vi "Material Theme Editor.vi"() -> ()   [LabVIEW 2021]
doc: "Import Material m3 JSON files to see the color scheme in LabVIEW.\n\nActions: +\n- Color Scheme: view and change colors for the theme mode +\n- Palette: see the palette color scales +\n- Text: see the text from the JSON file +\n- Buttons: see examples of the application to material button components - they can also be right clicked and copied so they can be directly pasted on an open front panel +\n\nOther options: +\n- Save the changes made in the editor (or save to a new file) +\n- Preview the theme on a lot of different front panel UI components +\n- See the overall colors of the palette and give ability to import into <i>User Colors</i>\n\n<b>Note:</b> if using the legacy XML files from earlier versions of the tool, they can be converted to the json format directly (assuming the original source doesn't exist still)\n\n<b>Code Developed By:</b> +\nDaniel Coons +\nTechnology Service Corporation +\nwww.tsc.com/atcs"
uses:
  Material Theme/Material Theme.lvclass
  _theme-editor/Theme Config/Theme Config.lvclass/Theme Config.ctl
  Material-Scheme/Material-Scheme.lvclass/Material-Scheme.ctl
  Material-Scheme/View-User Colors.vi
  Material-Scheme/Material-Scheme.lvclass
  Material-Palette/Material-Palette.lvclass
  user32.dll
  <vilib>/Utility/traverseref.llb/VI Scripting - Traverse.lvlib
  <vilib>/Utility/traverseref.llb/TRef TravTarget.ctl
  _theme-editor/Theme Config/Theme Config.lvclass
panel:
  in  "palette":bool
  in  "File Interaction":enum32{"load--buton", "convert--buton"}(radio)
  in  "tabs":enum32{"color", "palette", "json", "buttons"}(radio)
  in  "preview":bool
  in  "close":bool
  out "header":bool
  in  "save":bool
  in  "Theme Mode":u16(ring) items=["Light Theme", "Light Medium Contrast", "Light High Contrast", "Dark Theme", "Dark Medium Contrast", "Dark High Constrast"]
  in  "Tab Control":T1(tab)
  out "material JSON output":string
  in  "Color Level":u16(ring) items=["Primary", "Secondary", "Tertiary", "Error", "Primary Fixed", "Secondary Fixed", "Tertiary Fixed"]
  in  "Tab Control file":enum32{"load", "convert"}(tab)
  in  "json file path":path caption="Material Theme JSON File"
  in  "LabVIEW material theme":path
  # "Load a JSON M3 theme file from Google to \nview and edit the scheme."
  # "Can be generated through Figma or at:   https://material-foundation.github.io/material-theme-builder/<Material Website>"
  # "Load a TSC Material Theme legacy XML file to see modes\nand palette colors and convert to JSON format for long-term\nsupport."
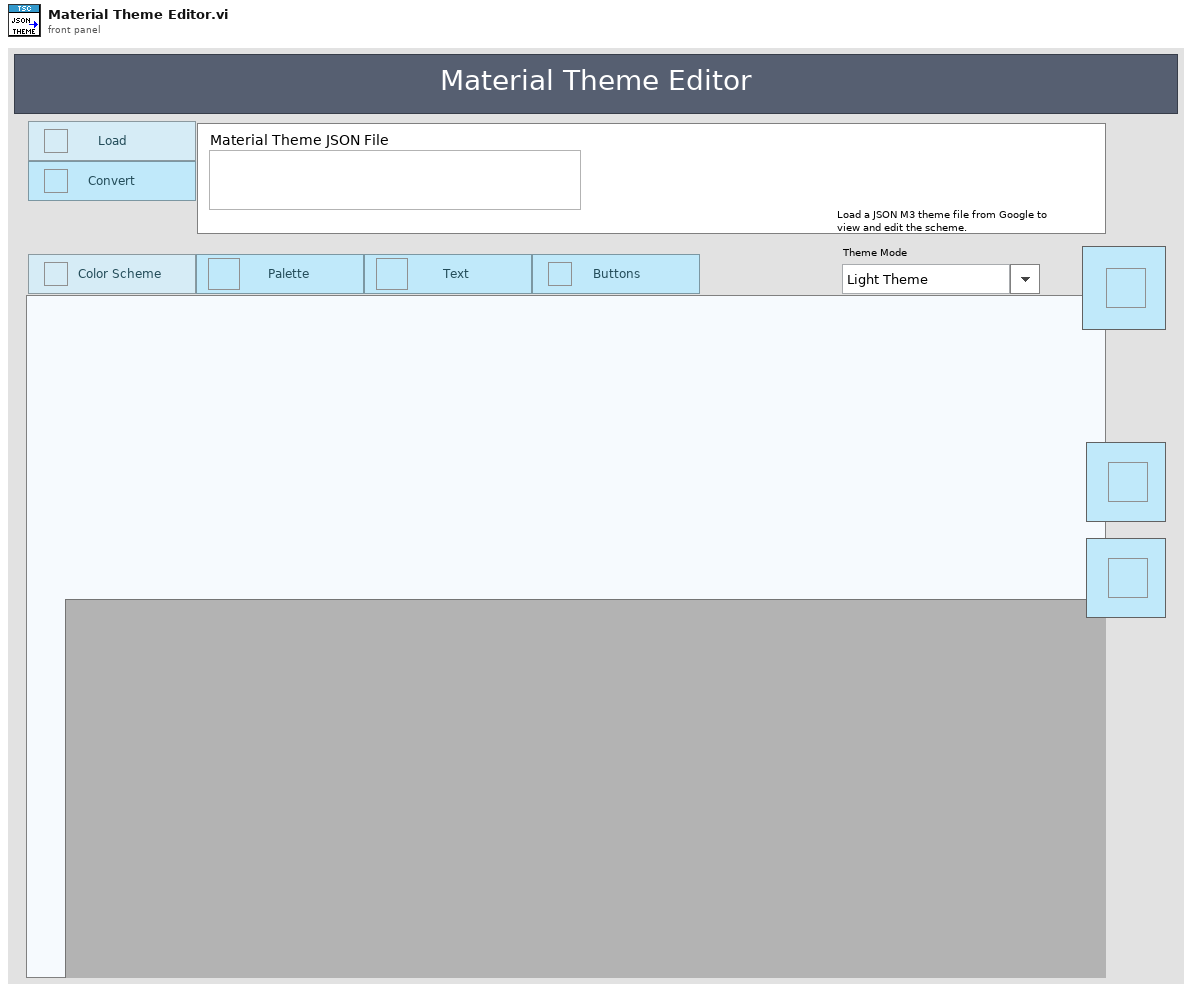
[diagram p1: front panel]
types:
  T1 = enum32{"Color Scheme", "Palette Variations", "JSON String", "buttons"}
  T2 = typedef "TRef TravTarget.ctl" = enum16{"FP", "BD", "Other"}
  T3 = enum16{"open", "replace", "create", "open or create", "replace or create", "replace or create with confirmation"}
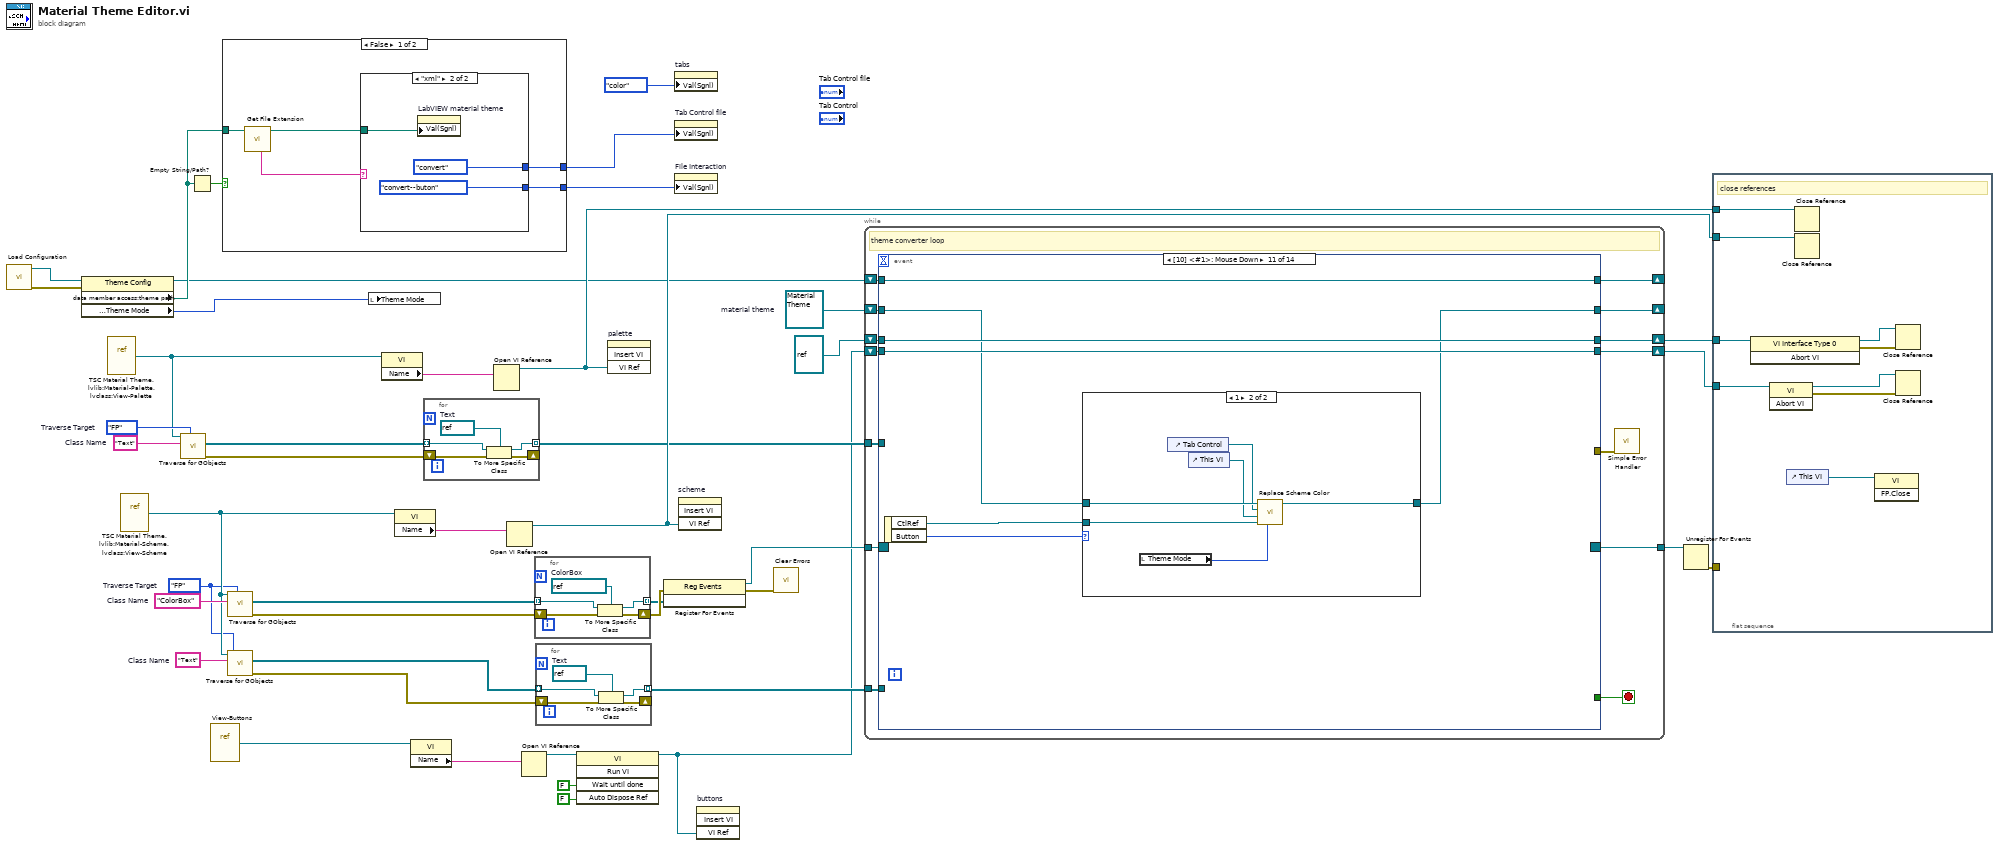
[diagram p0: block diagram]
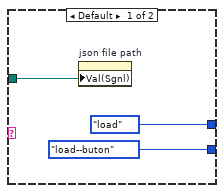
[diagram p2: hidden frame]
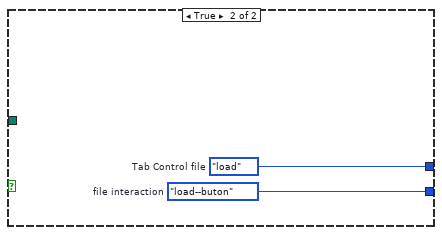
[diagram p3: hidden frame]
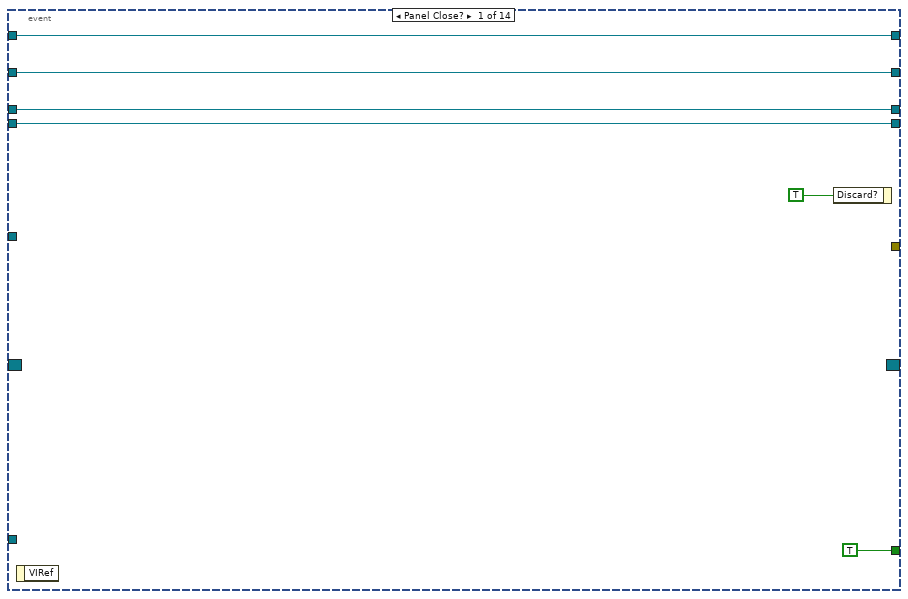
[diagram p4: hidden frame]
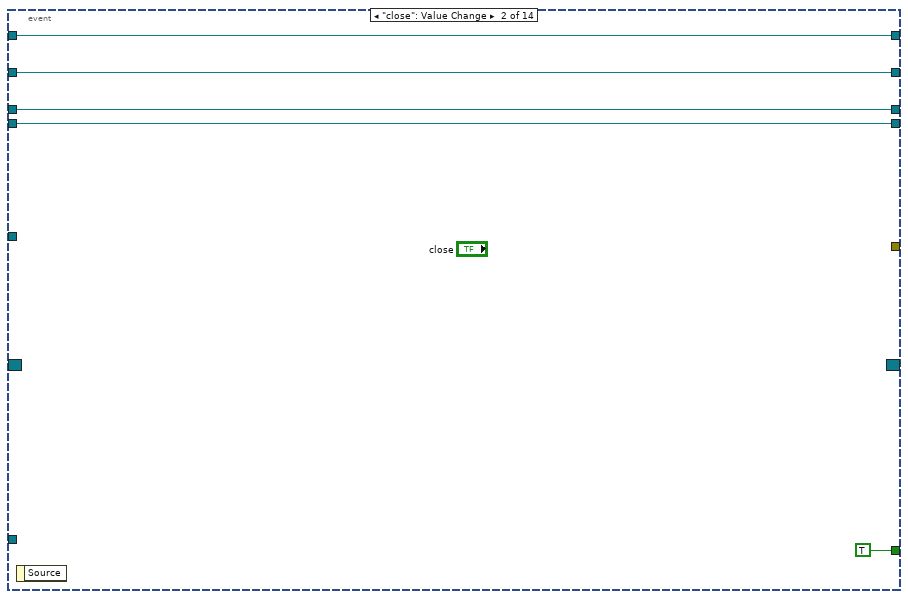
[diagram p5: hidden frame]
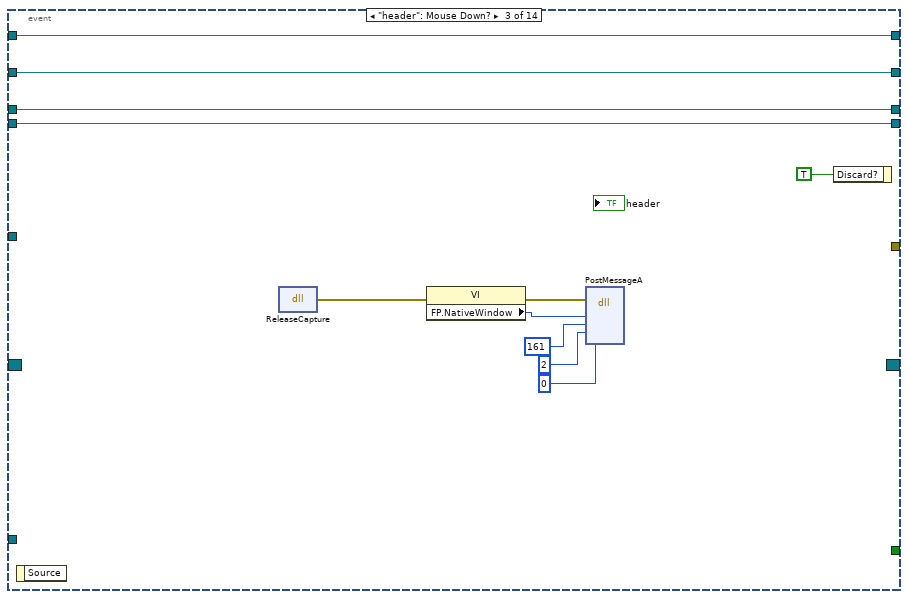
[diagram p6: hidden frame]
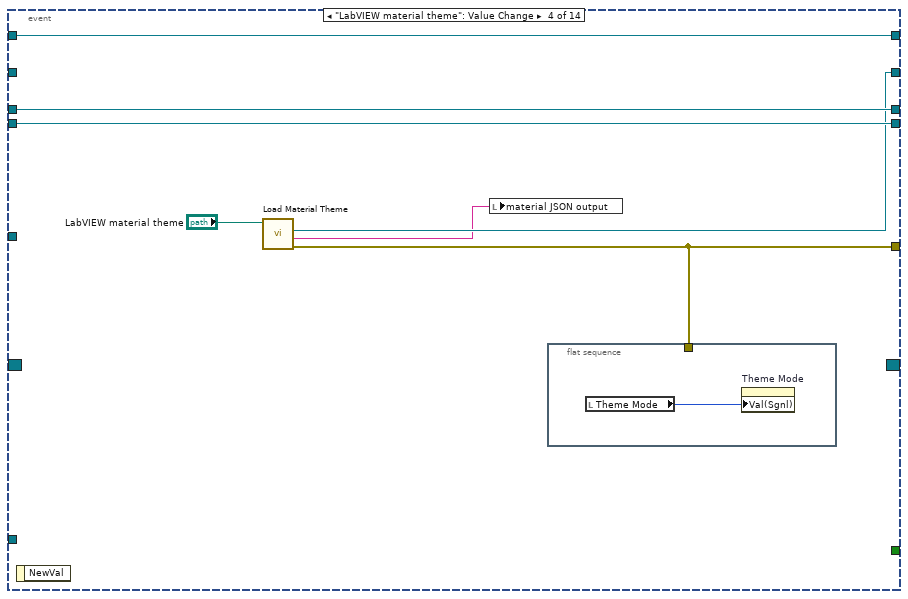
[diagram p7: hidden frame]
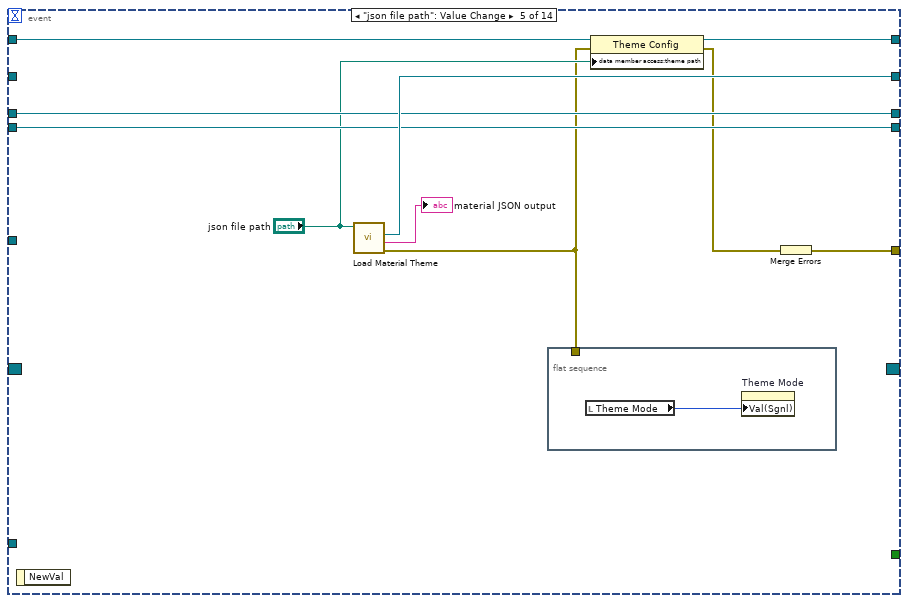
[diagram p8: hidden frame]
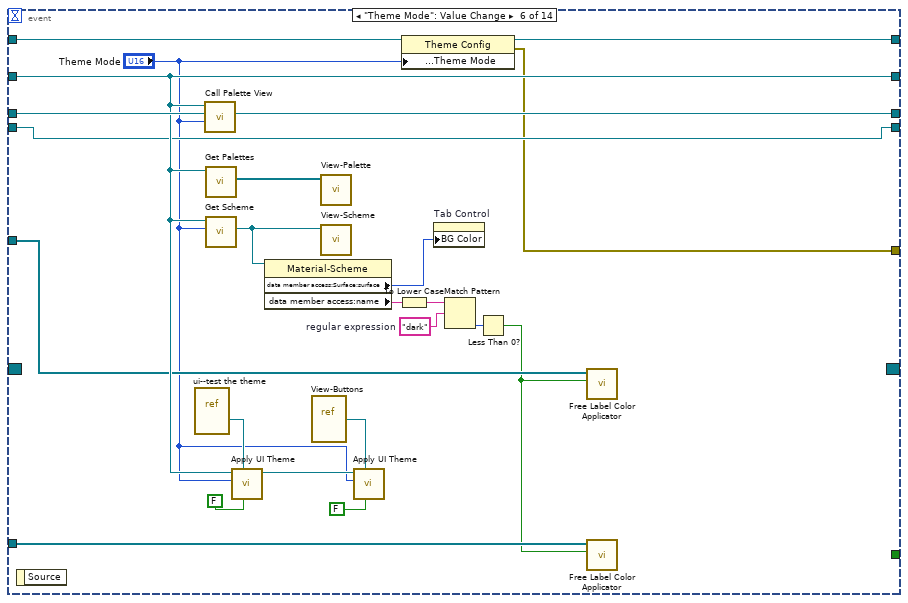
[diagram p9: hidden frame]
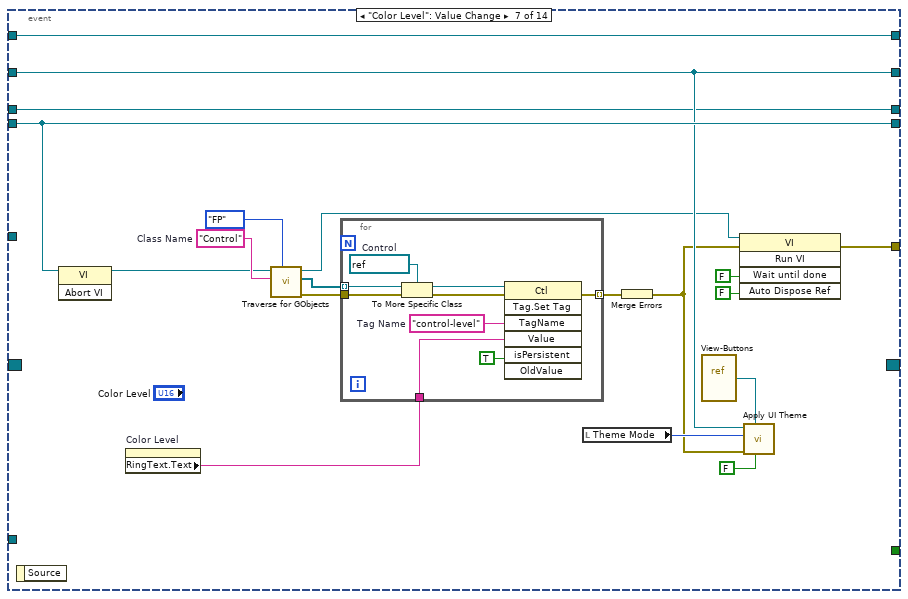
[diagram p10: hidden frame]
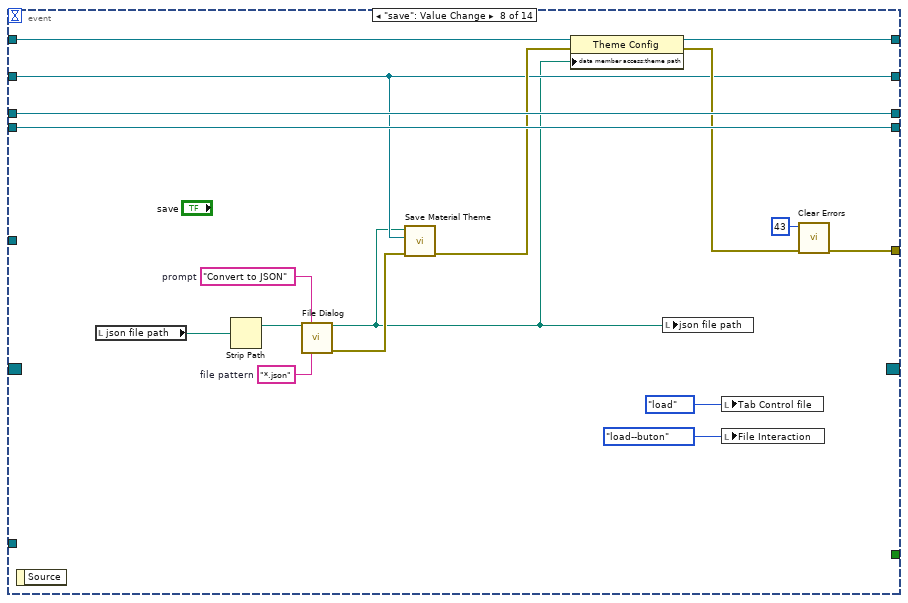
[diagram p11: hidden frame]
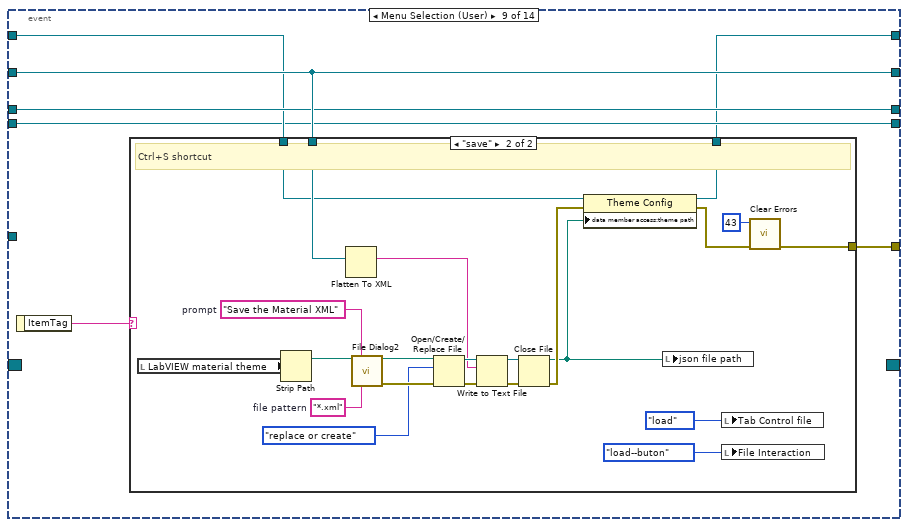
[diagram p12: hidden frame]
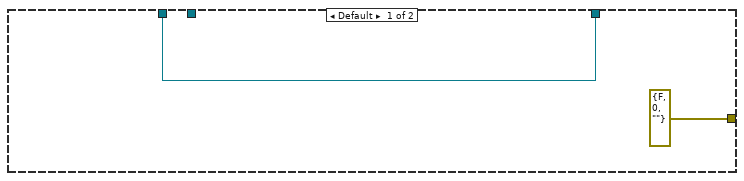
[diagram p13: hidden frame]
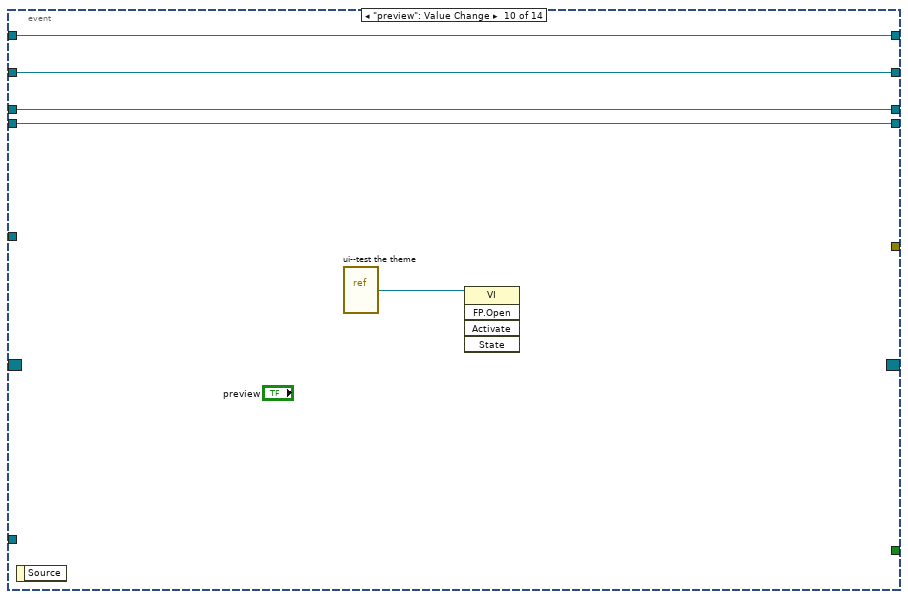
[diagram p14: hidden frame]
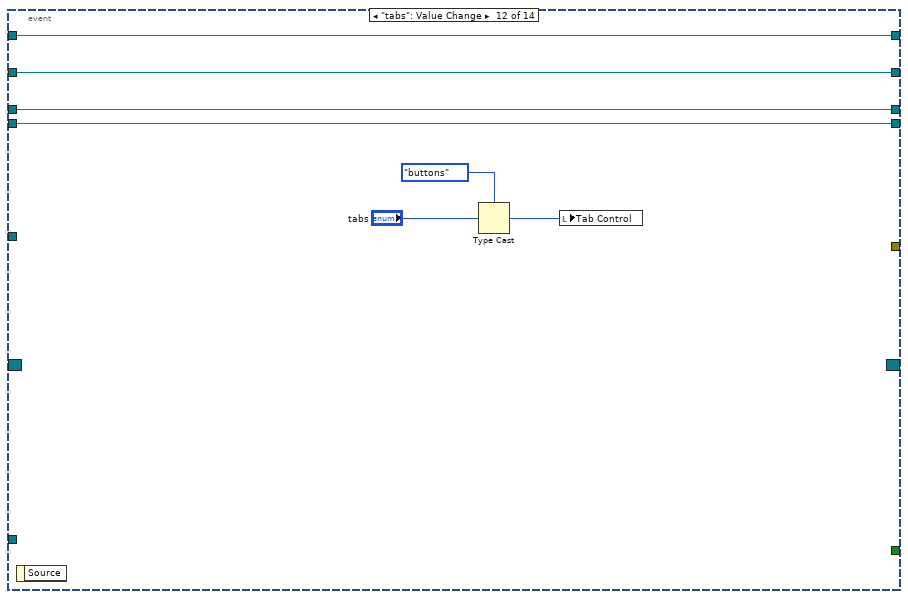
[diagram p16: hidden frame]
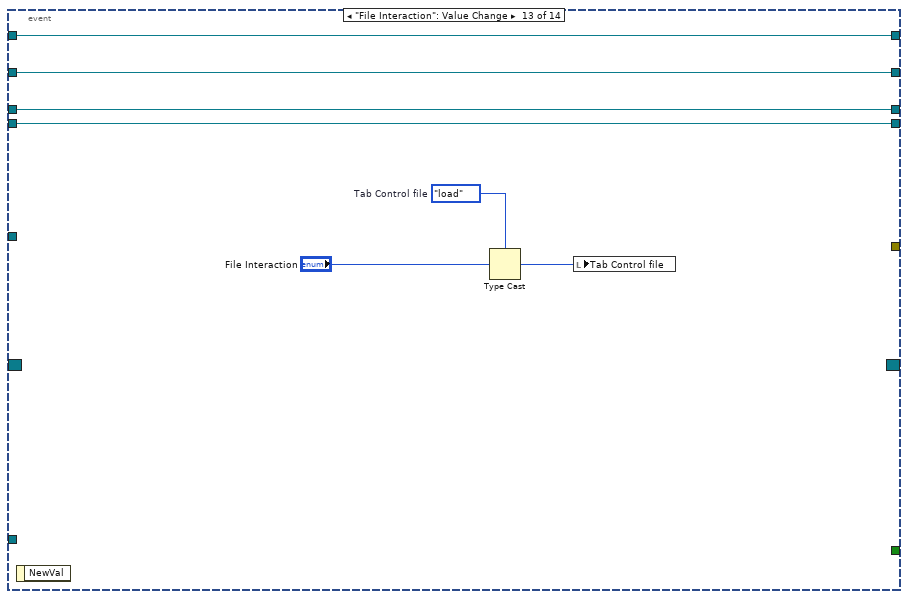
[diagram p17: hidden frame]
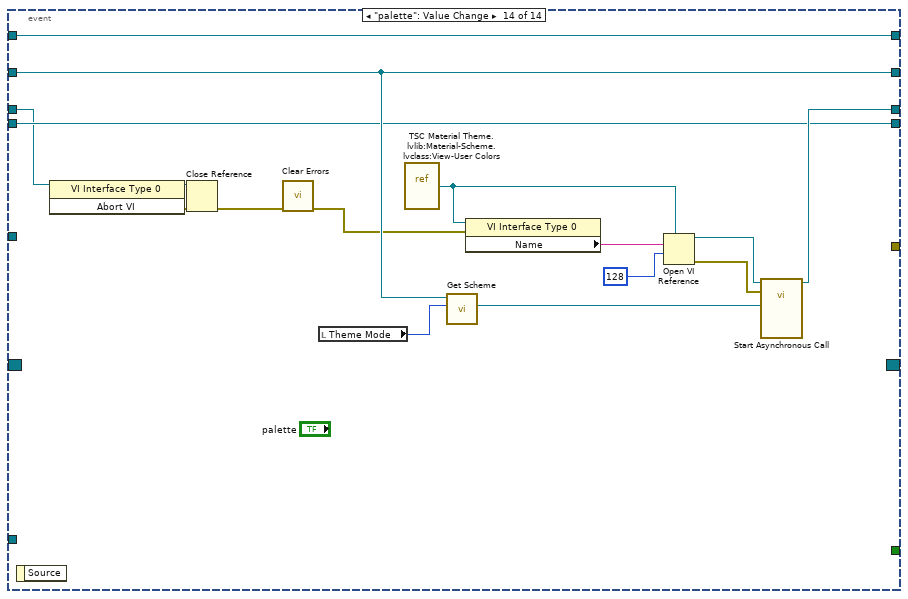
[diagram p18: hidden frame]
diagram:
  w24 = "Text"  # Class Name
  w27 = "Text"  # Class Name
  w28 = TRef_TravTarget."FP"  # Traverse Target
  w30 = refnum<class "Material Theme.lvclass"> refnum  # material theme
  w36 = "ColorBox"  # Class Name
  w22 = TRef_TravTarget."FP"  # Traverse Target
  n1 = call "Load Configuration.vi"() -> ("error out"=w10:errorcluster, "Theme Config out"=w9:refnum<class "Theme Config.lvclass">)  [unwired: 10 in]
  n2 = property class="Theme Config"(reference=w9, error in=w10) -> (reference out=w6:refnum<class "Theme Config.lvclass">, "data member access:theme path"=w8:path, "data member access:Theme Mode"=w3:u16)  [unwired: 1 out]
  n3 = vi-ref "TSC Material Theme.lvlib:Material-Palette.lvclass:View-Palette.vi"() -> (w7:refnum<vi>)
  n4 = vi-ref "TSC Material Theme.lvlib:Material-Scheme.lvclass:View-Scheme.vi"() -> (w23:refnum<vi>)
  n5 = call <vilib>:"Traverse for GObjects.vi"("Traverse Target"=w28, "Class Name"=w27, "VI Refnum"=w7) -> ("error out"=w41:errorcluster, "References"=w26:refnum<vi>[])  [unwired: 5 in, 2 out]
  n6 = Empty String/Path?(string/path=w8) -> (empty?=w29:bool)
  n7 = vi-ref "View-Buttons.vi"() -> (w17:refnum<vi>)
  n8 = case shown="False" w29 {
    tunnel: w8 -> [w49 _]
    tunnel: [w48 w56] -> w2
    tunnel: [w47 w57] -> w1
    frame False {
      n9 = call <vilib>:"Get File Extension.vi"("file"=w49) -> ("dup file"=w46:path, "unmodified file extension"=w45:string)  [unwired: 6 in, 3 out]
      n10 = case shown="\"xml\"" w45 {
        tunnel: w46 -> [w52 w55]
        tunnel: [enum32{"load--buton", "convert--buton"}."load--buton" ("Value (Signaling)") enum32{"load--buton", "convert--buton"}."convert--buton" ("Value (Signaling)")] -> w48
        tunnel: [enum32{"load", "convert"}."load" ("Tab Control file") enum32{"load", "convert"}."convert" ("Tab Control file")] -> w47
        frame Default {
          n11 = property on="json file path" class="Path"("Val(Sgnl)"=w52) -> ()  [unwired: 2 in, 2 out]
        }
        frame "xml" {
          n12 = property on="LabVIEW material theme" class="Path"("Val(Sgnl)"=w55) -> ()  [unwired: 2 in, 2 out]
        }
      }
    }
    frame True {
      w56 = enum32{"load--buton", "convert--buton"}."load--buton"  # file interaction
      w57 = enum32{"load", "convert"}."load"  # Tab Control file
    }
  }
  n13 = call <vilib>:"Traverse for GObjects.vi"("Traverse Target"=w22, "Class Name"=w36, "VI Refnum"=w23) -> ("error out"=w44:errorcluster, "References"=w34:refnum<vi>[])  [unwired: 5 in, 2 out]
  n14 = call <vilib>:"Traverse for GObjects.vi"("Traverse Target"=w22, "Class Name"=w24, "VI Refnum"=w23) -> ("error out"=w40:errorcluster, "References"=w21:refnum<vi>[])  [unwired: 5 in, 2 out]
  n15 = local write "Theme Mode"(w3) -> ()
  n16 = property class="VI"(reference=w7) -> ("Name"=w39:string)  [unwired: 1 in, 2 out]
  n17 = property class="VI"(reference=w23) -> ("Name"=w38:string)  [unwired: 1 in, 2 out]
  n18 = property class="VI"(reference=w17) -> ("Name"=w16:string)  [unwired: 1 in, 2 out]
  n19 = for {
    tunnel: w26 -> [w59] mode=indexing
    shift-right: [w61] -> _
    shift-left: w41 -> [w62]
    tunnel: [w58] -> w25 mode=indexing
    w60 = refnum<vi> refnum  # Text
    n20 = To More Specific Class(target class=w60, reference=w59, error in=w62) -> (specific class reference=w58:refnum<vi>, error out=w61:errorcluster)
  }
  n21 = Open VI Reference(vi path=w39) -> (vi reference=w37:refnum<vi>)  [unwired: 5 in, 1 out]
  n22 = Open VI Reference(vi path=w38) -> (vi reference=w33:refnum<vi>)  [unwired: 5 in, 1 out]
  n23 = Open VI Reference(vi path=w16) -> (vi reference=w18:refnum<vi>)  [unwired: 5 in, 1 out]
  n24 = for {
    tunnel: w34 -> [w64] mode=indexing
    shift-right: [w66] -> w43
    shift-left: w44 -> [w67]
    tunnel: [w63] -> w32 mode=indexing
    w65 = refnum<vi> refnum  # ColorBox
    n25 = To More Specific Class(target class=w65, reference=w64, error in=w67) -> (specific class reference=w63:refnum<vi>, error out=w66:errorcluster)
  }
  n26 = for {
    tunnel: w21 -> [w69] mode=indexing
    shift-right: [w71] -> _
    shift-left: w40 -> [w72]
    tunnel: [w68] -> w20 mode=indexing
    w70 = refnum<vi> refnum  # Text
    n27 = To More Specific Class(target class=w70, reference=w69, error in=w72) -> (specific class reference=w68:refnum<vi>, error out=w71:errorcluster)
  }
  n28 = invoke class="VI" method="Run VI"(reference=w18, "Wait until done"=FALSE ("Wait Until Done"), "Auto Dispose Ref"=FALSE ("Auto Dispose Reference")) -> (reference out=w13:refnum<vi>)  [unwired: 2 in, 4 out]
  n29 = invoke on="palette" class="SubPnl" method="Insert VI"("VI Ref"=w37) -> ()  [unwired: 3 in, 4 out]
  n30 = register-events(error in=w43, w32) -> (reference out=w35:refnum<event-registration>, error out=w42:errorcluster)  [unwired: 1 in]
  n31 = property on="tabs" class="RadioBtnsControl (strict)"("Val(Sgnl)"=enum32{"color", "palette", "json", "buttons"}."color" ("Value (Signaling)")) -> ()  [unwired: 2 in, 2 out]
  n32 = property on="Tab Control file" class="TabCtl (strict)"("Val(Sgnl)"=w1) -> ()  [unwired: 2 in, 2 out]
  n33 = property on="File Interaction" class="RadioBtnsControl (strict)"("Val(Sgnl)"=w2) -> ()  [unwired: 2 in, 2 out]
  n34 = invoke on="scheme" class="SubPnl" method="Insert VI"("VI Ref"=w33) -> ()  [unwired: 3 in, 4 out]
  n35 = invoke on="buttons" class="SubPnl" method="Insert VI"("VI Ref"=w13) -> ()  [unwired: 3 in, 4 out]
  n36 = call <vilib>:"Clear Errors.vi"("error in (no error)"=w42) -> ()  [unwired: 5 in, 2 out]
  n37 = while {
    shift-right: [w84] -> _
    shift-left: w30 -> [w83]
    tunnel: w35 -> [w82]
    tunnel: [w81] -> w31
    tunnel: w25 -> [w80]
    tunnel: w20 -> [w79]
    shift-right: [w77] -> w12
    shift-left: refnum<vi> refnum -> [w76]
    shift-right: [w74] -> _
    shift-left: w6 -> [w75]
    shift-right: [w73] -> w4
    shift-left: w13 -> [w78]
    stop <- w85 stop-if-true
    # "theme converter loop"
    n38 = event shown="[10] <#1>: Mouse Down" {
      selector: w82 -> [_ _ _ _ _ _ _ _ _ _ _ _ _ _]
      dyn-events: [_ _ _ _ _ _ _ _ _ _ _ _ _ _] -> w81
      timeout: _ -> [_ _ _ _ _ _ _ _ _ _ _ _ _ _]
      tunnel: [TRUE TRUE _ _ _ _ _ _ _ _ _ _ _ _] -> w85
      tunnel: [w90 w97 w101 w110 w125 w137 w156 w182 w201 w231 w232 w252 w258 w275] -> w84
      tunnel: w83 -> [w90 w97 w101 _ _ w137 w156 w182 w201 w231 w233 w252 w258 w275]
      tunnel: [_ _ _ w111 w126 w128 w162 w185 w202 _ _ _ _ _] -> w86
      tunnel: w80 -> [_ _ _ _ _ w132 _ _ _ _ _ _ _ _]
      tunnel: w79 -> [_ _ _ _ _ w141 _ _ _ _ _ _ _ _]
      tunnel: w78 -> [w87 w93 w98 w113 w122 w133 w167 w187 w197 w227 w235 w246 w255 w265]
      tunnel: [w89 w95 w100 w115 w124 w136 w152 w190 w199 w229 w237 w248 w257 w267] -> w77
      tunnel: w76 -> [w89 w95 w100 w115 w124 w138 w152 w190 w199 w229 w237 w248 w257 w262]
      tunnel: w75 -> [w88 w94 w99 w114 w123 w134 w151 w189 w198 w228 w236 w247 w256 w266]
      tunnel: [w88 w94 w99 w114 w121 w130 w151 w188 w196 w228 w236 w247 w256 w266] -> w74
      tunnel: [w87 w93 w98 w113 w122 w133 w167 w187 w197 w227 w235 w246 w255 w265] -> w73
      event Panel Close? {
        n39 = event-data() -> ()  [unwired: 1 in, 1 out]
        n40 = event-data("Discard?"=TRUE) -> ()  [unwired: 1 in, 1 out]
      }
      event "close": Value Change {
        n41 = event-data() -> ()  [unwired: 1 in, 1 out]
      }
      event "header": Mouse Down? {
        n42 = event-data() -> ()  [unwired: 1 in, 1 out]
        n43 = dll-call lib="user32.dll" fn="ReleaseCapture"() -> (error out=w108:errorcluster)  [unwired: 4 in, 1 out]
        n44 = property class="VI"(error in=w108) -> (error out=w107:errorcluster, "FP.NativeWindow"=w102:u64)  [unwired: 1 in, 1 out]
        n45 = dll-call lib="user32.dll" fn="PostMessageA"(error in=w107, "hWnd"=w102, "Msg"=161, "wParam"=2, "lParam"=0) -> ()  [unwired: 7 in, 2 out]
        n46 = event-data("Discard?"=TRUE) -> ()  [unwired: 1 in, 1 out]
      }
      event "LabVIEW material theme": Value Change {
        n47 = event-data() -> ()  [unwired: 1 in, 1 out]
        n48 = call "Load Material Theme.vi"("file path"="LabVIEW material theme") -> ("error out"=w111:errorcluster, "text"=w109:string, "Theme"=w110:refnum<class "Material Theme.lvclass">)  [unwired: 8 in]
        n49 = local write "material JSON output"(w109) -> ()
        n50 = flat-sequence {
          tunnel: w111 -> [_]
          frame #0 {
            n51 = local read "Theme Mode"() -> (w116:u16)
            n52 = property on="Theme Mode" class="Ring (strict)"("Val(Sgnl)"=w116) -> ()  [unwired: 2 in, 2 out]
          }
        }
      }
      event "json file path": Value Change {
        n53 = event-data() -> ()  [unwired: 1 in, 1 out]
        n54 = call "Load Material Theme.vi"("file path"="json file path") -> ("error out"=w119:errorcluster, "text"=→"material JSON output":string, "Theme"=w125:refnum<class "Material Theme.lvclass">)  [unwired: 8 in]
        n55 = flat-sequence {
          tunnel: w119 -> [_]
          frame #0 {
            n56 = local read "Theme Mode"() -> (w127:u16)
            n57 = property on="Theme Mode" class="Ring (strict)"("Val(Sgnl)"=w127) -> ()  [unwired: 2 in, 2 out]
          }
        }
        n58 = property class="Theme Config"(reference=w123, error in=w119, "data member access:theme path"="json file path") -> (reference out=w121:refnum<class "Theme Config.lvclass">, error out=w118:errorcluster)
        n59 = Merge Errors(w118) -> (w126:errorcluster)
      }
      event "Theme Mode": Value Change {
        w144 = "dark"  # regular expression
        n60 = event-data() -> ()  [unwired: 1 in, 1 out]
        n61 = vi-ref "ui--test the theme.vi"() -> (w149:refnum<vi>)
        n62 = call "Call Palette View.vi"("Theme Mode"="Theme Mode", "VI ref in"=w138, "Material Theme"=w137) -> ("VI ref"=w136:refnum<vi>)  [unwired: 7 in, 1 out]
        n63 = call "Get Palettes.vi"("Material Theme in"=w137) -> ("Material-Palettes"=w150:refnum<class "Material-Palette.lvclass">[])  [unwired: 8 in, 2 out]
        n64 = call "Get Scheme.vi"("Theme"="Theme Mode", "Material Theme in"=w137) -> ("Material-Scheme"=w147:refnum<class "Material-Scheme.lvclass">)  [unwired: 7 in, 2 out]
        n65 = call "Apply UI Theme.vi"("save?"=FALSE, "VI Refnum"=w149, "Theme Mode"="Theme Mode", "Material Theme in"=w137) -> ("Material Theme out"=w135:refnum<class "Material Theme.lvclass">)  [unwired: 6 in, 1 out]
        n66 = property class="Material-Scheme"(reference=w147) -> ("data member access:Surface:surface"=w146:u32, "data member access:name"=w145:string)  [unwired: 1 in, 2 out]
        n67 = vi-ref "View-Buttons.vi"() -> (w139:refnum<vi>)
        n68 = call "View-Palette.vi"("Array"=w150) -> ()  [unwired: 11 in]
        n69 = call "View-Scheme.vi"("Material-Scheme.lvclass"=w147) -> ()  [unwired: 11 in]
        n70 = call "Apply UI Theme.vi"("save?"=FALSE, "VI Refnum"=w139, "Theme Mode"="Theme Mode", "Material Theme in"=w135) -> ()  [unwired: 6 in, 2 out]
        n71 = To Lower Case(string=w145) -> (all lower case string=w143:string)
        n72 = property class="Theme Config"(reference=w134, "data member access:Theme Mode"="Theme Mode") -> (reference out=w130:refnum<class "Theme Config.lvclass">, error out=w128:errorcluster)  [unwired: 1 in]
        n73 = property on="Tab Control" class="TabCtl (strict)"("BG Color"=w146) -> ()  [unwired: 2 in, 2 out]
        n74 = Match Pattern(string=w143, regular expression=w144) -> (offset past match=w142:i32)  [unwired: 1 in, 3 out]
        n75 = Less Than 0?(x=w142) -> (x < 0?=w131:bool)
        n76 = call "Free Label Color Applicator.vi"("Dark Text?"=w131, "Text Labels"=w132) -> ()  [unwired: 10 in]
        n77 = call "Free Label Color Applicator.vi"("Dark Text?"=w131, "Text Labels"=w141) -> ()  [unwired: 10 in]
      }
      event "Color Level": Value Change {
        w169 = "Control"  # Class Name
        n78 = event-data() -> ()  [unwired: 1 in, 1 out]
        n79 = invoke class="VI" method="Abort VI"(reference=w167) -> (reference out=w161:refnum<vi>)  [unwired: 2 in, 2 out]
        n80 = property on="Color Level" class="Ring (strict)"() -> ("RingText.Text"=w164:string)  [unwired: 2 in, 2 out]
        n81 = call <vilib>:"Traverse for GObjects.vi"("Traverse Target"=TRef_TravTarget."FP", "Class Name"=w169, "VI Refnum"=w161) -> ("error out"=w165:errorcluster, "References"=w166:refnum<vi>[], "dup VI Refnum"=w153:refnum<vi>)  [unwired: 5 in, 1 out]
        n82 = for {
          tunnel: w166 -> [w177] mode=indexing
          tunnel: w165 -> [w176]
          tunnel: w164 -> [w172]
          tunnel: [w170] -> w163 mode=indexing
          w175 = refnum<vi> refnum  # Control
          w178 = "control-level"  # Tag Name
          n83 = To More Specific Class(target class=w175, reference=w177, error in=w176) -> (specific class reference=w173:refnum<vi>, error out=w174:errorcluster)
          n84 = invoke class="Ctl" method="Tag.Set Tag"(reference=w173, error in=w174, "TagName"=w178, "Value"=w172, "isPersistent"=TRUE ("Is Persistent?")) -> (error out=w170:errorcluster)  [unwired: 2 in, 6 out]
        }
        n85 = local read "Theme Mode"() -> (w155:u16)
        n86 = Merge Errors(w163) -> (w154:errorcluster)
        n87 = vi-ref "View-Buttons.vi"() -> (w158:refnum<vi>)
        n88 = invoke class="VI" method="Run VI"(reference=w153, error in=w154, "Wait until done"=FALSE ("Wait Until Done"), "Auto Dispose Ref"=FALSE ("Auto Dispose Reference")) -> (error out=w162:errorcluster)  [unwired: 1 in, 4 out]
        n89 = call "Apply UI Theme.vi"("save?"=FALSE, "VI Refnum"=w158, "error in"=w154, "Theme Mode"=w155, "Material Theme in"=w156) -> ()  [unwired: 5 in, 2 out]
      }
      event "save": Value Change {
        w191 = "Convert to JSON"  # prompt
        w194 = "*.json"  # file pattern
        n90 = event-data() -> ()  [unwired: 1 in, 1 out]
        n91 = local read "json file path"() -> (w193:path)
        n92 = Strip Path(path=w193) -> (stripped path=w192:path)  [unwired: 1 out]
        n93 = call "File Dialog"("start path"=w192, "prompt"=w191, "pattern (all files)"=w194) -> ("selected path"=w181:path, "error out"=w184:errorcluster)  [unwired: 9 in, 2 out]
        n94 = call "Save Material Theme.vi"("error in"=w184, "Theme"=w182, "file path"=w181) -> ("error out"=w183:errorcluster)  [unwired: 7 in, 1 out]
        n95 = property class="Theme Config"(reference=w189, error in=w183, "data member access:theme path"=w181) -> (reference out=w188:refnum<class "Theme Config.lvclass">, error out=w186:errorcluster)
        n96 = local write "json file path"(w181) -> ()
        n97 = local write "Tab Control file"(enum32{"load", "convert"}."load" ("Tab Control file")) -> ()
        n98 = local write "File Interaction"(enum32{"load--buton", "convert--buton"}."load--buton" ("Value (Signaling)")) -> ()
        n99 = call <vilib>:"Clear Errors.vi"("error in (no error)"=w186, "specific error code to clear (0: all)"=43) -> ("error out"=w185:errorcluster)  [unwired: 4 in, 1 out]
      }
      event Menu Selection (User) {
        n100 = event-data() -> ("ItemTag"=w200:string)  [unwired: 1 in]
        n101 = case shown="\"save\"" w200 {
          tunnel: w201 -> [_ w223]
          tunnel: [errorcluster {"status"=FALSE, "code"=0, "source"=""} ("error out") w207] -> w202
          tunnel: w198 -> [w203 w212]
          tunnel: [w203 w211] -> w196
          frame Default {
          }
          frame "save" {
            w216 = "Save the Material XML"  # prompt
            w215 = "*.xml"  # file pattern
            # "Ctrl+S shortcut"
            n102 = local read "LabVIEW material theme"() -> (w218:path)
            n103 = Strip Path(path=w218) -> (stripped path=w217:path)  [unwired: 1 out]
            n104 = Flatten To XML(6:w223) -> (2:w213:string)
            n105 = call "File Dialog2"("start path"=w217, "prompt"=w216, "pattern (all files)"=w215) -> ("selected path"=w219:path, "error out"=w224:errorcluster)  [unwired: 9 in, 2 out]
            n106 = Open/Create/Replace File(file path (use dialog)=w219, error in=w224, operation (0:open)=T3."replace or create") -> (refnum out=w221:refnum<file>, error out=w225:errorcluster)  [unwired: 3 in, 1 out]
            n107 = Write to Text File(file (use dialog)=w221, text=w213, error in=w225) -> (refnum out=w220:refnum<file>, error out=w226:errorcluster)  [unwired: 1 in, 1 out]
            n108 = Close File(refnum=w220, error in=w226) -> (path=w209:path, error out=w210:errorcluster)
            n109 = property class="Theme Config"(reference=w212, error in=w210, "data member access:theme path"=w209) -> (reference out=w211:refnum<class "Theme Config.lvclass">, error out=w208:errorcluster)
            n110 = local write "json file path"(w209) -> ()
            n111 = local write "Tab Control file"(enum32{"load", "convert"}."load" ("Tab Control file")) -> ()
            n112 = local write "File Interaction"(enum32{"load--buton", "convert--buton"}."load--buton" ("Value (Signaling)")) -> ()
            n113 = call <vilib>:"Clear Errors.vi"("error in (no error)"=w208, "specific error code to clear (0: all)"=43) -> ("error out"=w207:errorcluster)  [unwired: 4 in, 1 out]
          }
        }
      }
      event "preview": Value Change {
        n114 = event-data() -> ()  [unwired: 1 in, 1 out]
        n115 = vi-ref "ui--test the theme.vi"() -> (w230:refnum<vi>)
        n116 = invoke class="VI" method="FP.Open"(reference=w230) -> ()  [unwired: 4 in, 5 out]
      }
      event Mouse Down {
        n117 = event-data() -> ("CtlRef"=w238:refnum<vi>, "Button"=w234:u16)  [unwired: 1 in]
        n118 = case shown="1" w234 {
          tunnel: w238 -> [_ w242]
          tunnel: w233 -> [w239 w245]
          tunnel: [w239 w244] -> w232
          frame 0, Default {
          }
          frame 1 {
            n119 = local read "Theme Mode"() -> (w243:u16)
            n120 = control-ref of="Tab Control"() -> (w241:refnum<vi>)
            n121 = control-ref of="This VI"() -> (w240:refnum<vi>)
            n122 = call "Replace Scheme Color.vi"("Theme Mode"=w243, "Colorbox ref in"=w242, "This VI"=w240, "TabControl in"=w241, "Material Theme in"=w245) -> ("Material Theme out"=w244:refnum<class "Material Theme.lvclass">)  [unwired: 6 in]
          }
        }
      }
      event "tabs": Value Change {
        n123 = event-data() -> ()  [unwired: 1 in, 1 out]
        n124 = Type Cast(type=T1."buttons" ("Tab Control"), x="tabs") -> (*(type *) &x=w249:T1)
        n125 = local write "Tab Control"(w249) -> ()
      }
      event "File Interaction": Value Change {
        w253 = enum32{"load", "convert"}."load"  # Tab Control file
        n126 = event-data() -> ()  [unwired: 1 in, 1 out]
        n127 = Type Cast(type=w253, x="File Interaction") -> (*(type *) &x=w254:enum32{"load", "convert"})
        n128 = local write "Tab Control file"(w254) -> ()
      }
      event "palette": Value Change {
        n129 = event-data() -> ()  [unwired: 1 in, 1 out]
        n130 = invoke class="VI Interface Type 0" method="Abort VI"(reference=w262) -> (reference out=w261:refnum<vi>, error out=w260:errorcluster)  [unwired: 2 in, 1 out]
        n131 = Close Reference(reference=w261, error in (no error)=w260) -> (error out=w264:errorcluster)
        n132 = call <vilib>:"Clear Errors.vi"("error in (no error)"=w264) -> ("error out"=w263:errorcluster)  [unwired: 5 in, 1 out]
        n133 = local read "Theme Mode"() -> (w274:u16)
        n134 = vi-ref "TSC Material Theme.lvlib:Material-Scheme.lvclass:View-User Colors.vi"() -> (w269:refnum<vi>)
        n135 = call "Get Scheme.vi"("Theme"=w274, "Material Theme in"=w275) -> ("Material-Scheme"=w273:refnum<class "Material-Scheme.lvclass">)  [unwired: 7 in, 2 out]
        n136 = property class="VI Interface Type 0"(reference=w269, error in=w263) -> ("Name"=w272:string)  [unwired: 2 out]
        n137 = Open VI Reference(type specifier VI Refnum (for type only)=w269, vi path=w272, options=128) -> (vi reference=w270:refnum<vi>, error out=w268:errorcluster)  [unwired: 3 in]
        n138 = call-by-ref "Start Asynchronous Call"(reference=w270, error in=w268, "Material-Scheme.lvclass"=w273) -> (reference out=w267:refnum<vi>)  [unwired: 11 in, 1 out]
      }
    }
    n139 = call <vilib>:"Simple Error Handler.vi"("error in (no error)"=w86) -> ()  [unwired: 4 in, 5 out]
  }
  n140 = Unregister For Events(event registration refnum=w31) -> (error out=w5:errorcluster)  [unwired: 1 in]
  n141 = flat-sequence {
    tunnel: w37 -> [w284]
    tunnel: w33 -> [w283]
    tunnel: w12 -> [w278]
    tunnel: w5 -> [_]
    tunnel: w4 -> [w277]
    frame #0 {
      # "close references"
      n142 = invoke class="VI Interface Type 0" method="Abort VI"(reference=w278) -> (reference out=w279:refnum<vi>, error out=w280:errorcluster)  [unwired: 2 in, 1 out]
      n143 = invoke class="VI" method="Abort VI"(reference=w277) -> (reference out=w282:refnum<vi>, error out=w281:errorcluster)  [unwired: 2 in, 1 out]
      n144 = control-ref of="This VI"() -> (w276:refnum<vi>)
      n145 = Close Reference(reference=w284) -> ()  [unwired: 1 in, 1 out]
      n146 = Close Reference(reference=w283) -> ()  [unwired: 1 in, 1 out]
      n147 = invoke class="VI" method="FP.Close"(reference=w276) -> ()  [unwired: 2 in, 3 out]
      n148 = Close Reference(reference=w279, error in (no error)=w280) -> ()  [unwired: 1 out]
      n149 = Close Reference(reference=w282, error in (no error)=w281) -> ()  [unwired: 1 out]
    }
  }
